vi "MAIZE Offline Console.vi"() -> ()   [LabVIEW 2025]
doc: "Offline MAIZE operator console with modeled equipment and the shared controller."
panel:
  in  "End session":bool
  out "Cryo gate valve":picture
  out "Turbo gate valve":picture
  out "Let-up valve":picture
  out "Roughing valve":picture
  out "Latched faults":string
  out "Active interlocks":string
  out "Opening outputs":string
  out "Chamber pressure":string
  out "Operating state":string
  out "Model status":string
  in  "Test condition":T1(ring)
  in  "Mode":enum16{"OFF", "MANUAL", "AUTO"}(ring)=enum."OFF"
  in  "Close / Stop":bool
  in  "Vent Start":bool
  in  "Pumpdown":bool
  in  "Arm / Reset":bool
  in  "Cryo OPEN":bool
  in  "Turbo OPEN":bool
  in  "Let-up OPEN":bool
  in  "Roughing OPEN":bool
  # "MAIZE     /     OFFLINE SIMULATION"
  # "MAINTAINED VALVE REQUESTS"
  # "Roughing and Let-up show selector requests"
  # "Turbo and Cryo show modeled reed feedback"
  # "MODE AND MOMENTARY CONTROLS"
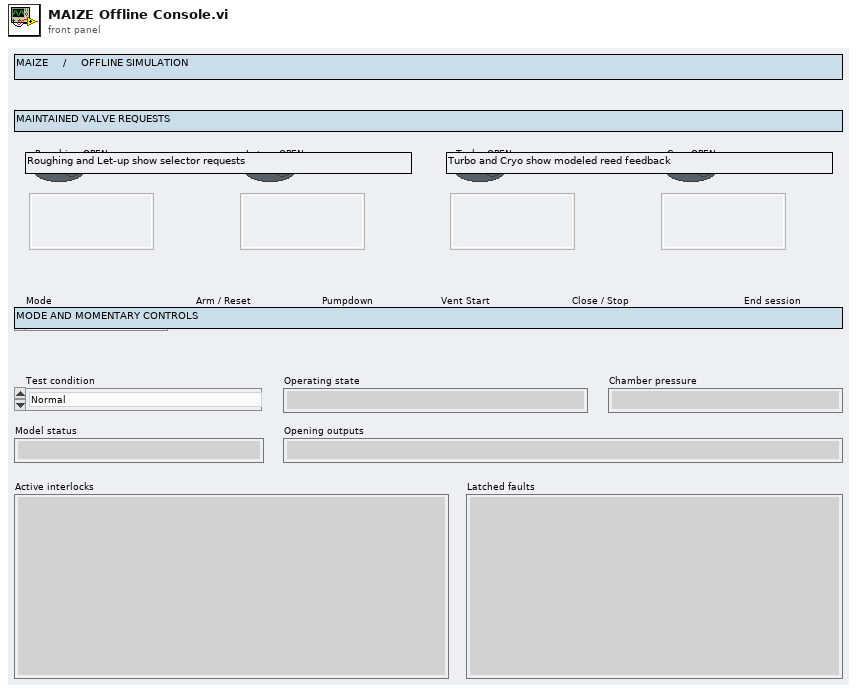
[diagram p1: front panel]
types:
  T1 = enum16{"Normal", "Pressure signal lost", "Actuator air lost", "Roughing pump not ready", "Cryopump not ready", "Turbo not at speed", "Turbo backing lost", "Filament ON", "Lab enable lost", "Coil-feed inhibit", "Vent process inhibit", "Turbo gate stuck", "Cryo gate stuck", "Turbo feedback conflict", "Cryo feedback conflict", "Panel inputs lost"}
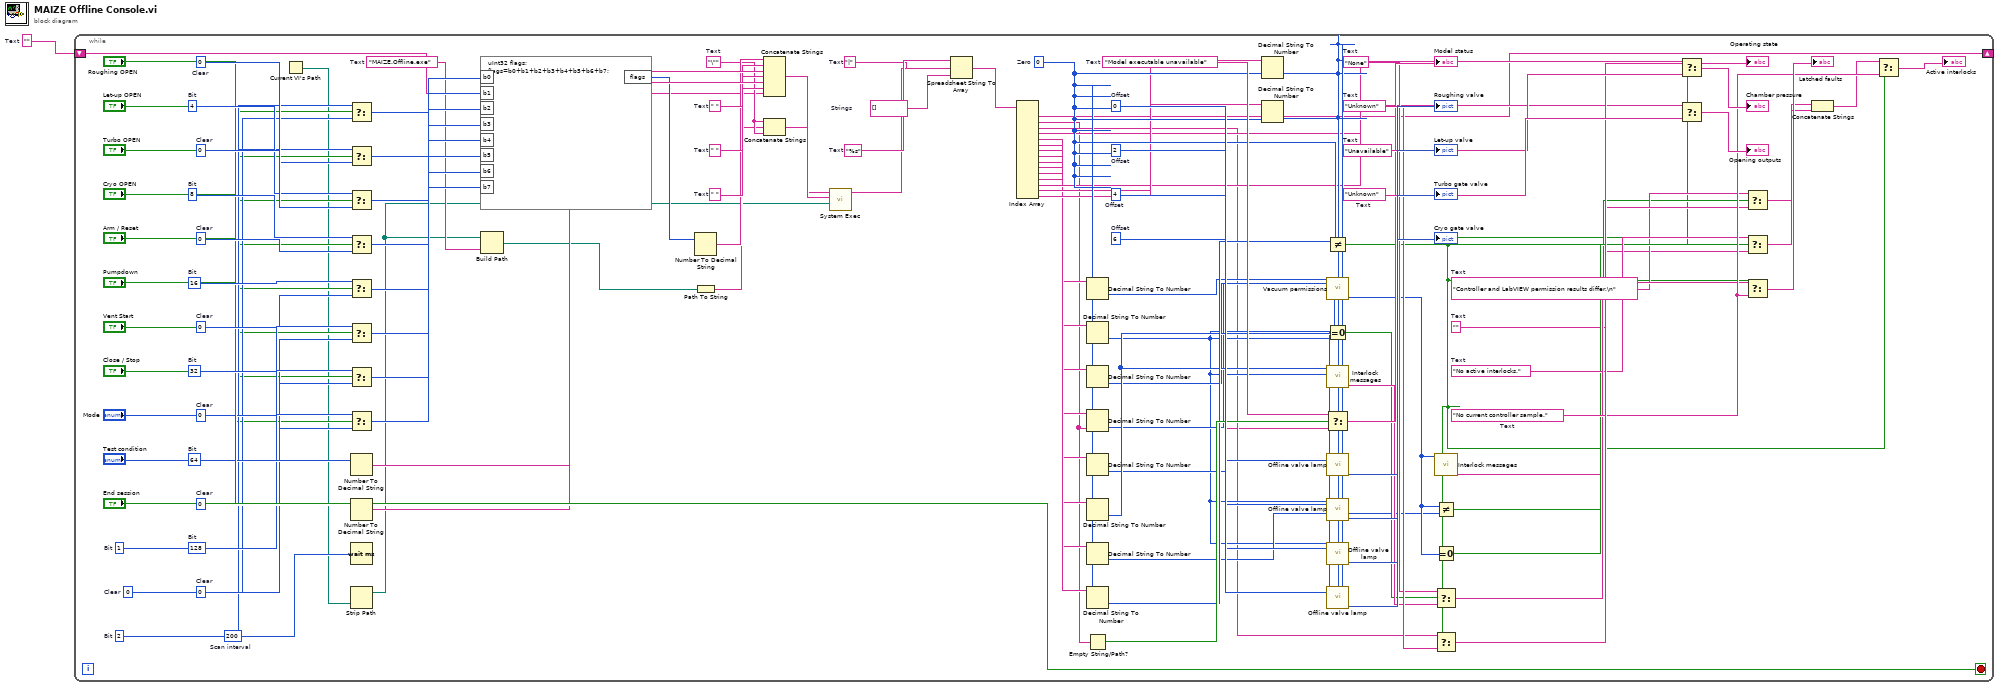
[diagram p0: block diagram]
diagram:
  w1 = ""  # Text
  n1 = while {
    shift-right: [w3] -> _
    shift-left: w1 -> [w2]
    stop <- "End session" stop-if-true
    w118 = u32 200  # Scan interval
    w116 = u32 6  # Offset
    w114 = u32 4  # Offset
    w112 = u32 2  # Offset
    w110 = u32 0  # Offset
    w104 = "Unknown"  # Text
    w102 = "Unavailable"  # Text
    w100 = "Unknown"  # Text
    w98 = "Model executable unavailable"  # Text
    w96 = "No current controller sample."  # Text
    w93 = "None"  # Text
    w89 = "No active interlocks."  # Text
    w86 = ""  # Text
    w85 = "Controller and LabVIEW permission results differ.\n"  # Text
    w72 = u32 0  # Zero
    w56 = "%s"  # Text
    w55 = string[] []  # Strings
    w54 = "|"  # Text
    w51 = " "  # Text
    w49 = " "  # Text
    w47 = " "  # Text
    w41 = u32 0  # Clear
    w40 = u32 128  # Bit
    w38 = u32 0  # Clear
    w37 = u32 64  # Bit
    w35 = u32 0  # Clear
    w34 = u32 32  # Bit
    w32 = u32 0  # Clear
    w31 = u32 16  # Bit
    w29 = u32 0  # Clear
    w28 = u32 8  # Bit
    w26 = u32 0  # Clear
    w25 = u32 4  # Bit
    w23 = u32 0  # Clear
    w22 = u32 2  # Bit
    w20 = u32 0  # Clear
    w19 = u32 1  # Bit
    w9 = "\""  # Text
    w6 = "MAIZE.Offline.exe"  # Text
    n2 = Current VI's Path() -> (path=w4:path)
    n3 = Select(t=w19, s="Roughing OPEN", f=w20) -> (s? t:f=w21:u32)
    n4 = Select(t=w22, s="Let-up OPEN", f=w23) -> (s? t:f=w24:u32)
    n5 = Select(t=w25, s="Turbo OPEN", f=w26) -> (s? t:f=w27:u32)
    n6 = Select(t=w28, s="Cryo OPEN", f=w29) -> (s? t:f=w30:u32)
    n7 = Select(t=w31, s="Arm / Reset", f=w32) -> (s? t:f=w33:u32)
    n8 = Select(t=w34, s="Pumpdown", f=w35) -> (s? t:f=w36:u32)
    n9 = Select(t=w37, s="Vent Start", f=w38) -> (s? t:f=w39:u32)
    n10 = Select(t=w40, s="Close / Stop", f=w41) -> (s? t:f=w42:u32)
    n11 = Number To Decimal String(number="Mode") -> (decimal integer string=w48:string)  [unwired: 1 in]
    n12 = Number To Decimal String(number="Test condition") -> (decimal integer string=w50:string)  [unwired: 1 in]
    n13 = Wait (ms)(milliseconds to wait=w118) -> ()  [unwired: 1 out]
    n14 = Strip Path(path=w4) -> (stripped path=w5:path)  [unwired: 1 out]
    n15 = formula code="uInt32 flags;\nflags=b0+b1+b2+b3+b4+b5+b6+b7;"("b0"=w21, "b1"=w24, "b2"=w27, "b3"=w30, "b4"=w33, "b5"=w36, "b6"=w39, "b7"=w42) -> ("flags"=w43:u32)
    n16 = Build Path(base path=w5, name or relative path=w6) -> (appended path=w7:path)
    n17 = Number To Decimal String(number=w43) -> (decimal integer string=w46:string)  [unwired: 1 in]
    n18 = Path To String(path=w7) -> (string=w8:string)
    n19 = Concatenate Strings(w46, w47, w48, w49, w50, w51, w2) -> (w52:string)
    n20 = Concatenate Strings(w9, w8, w9) -> (w10:string)
    n21 = call <vilib>:"System Exec.vi"("working directory"=w5, "standard input"=w52, "command line"=w10) -> ("standard output"=w53:string)  [unwired: 5 in, 3 out]
    n22 = Spreadsheet String To Array(delimiter (Tab)=w54, format string=w56, spreadsheet string=w53, array type (2D Dbl)=w55) -> (array=w57:string[])
    n23 = Index Array(array=w57) -> (element #1=w3:string, element #2=w58:string, element #3=w59:string, element #4=w60:string, element #5=w61:string, element #6=w62:string, element #7=w63:string, element #8=w64:string, element #9=w65:string, element #10=w66:string, element #11=w67:string, element #12=w68:string, element #13=w69:string, element #14=w70:string, element #15=w71:string)  [unwired: 15 in]
    n24 = Decimal String To Number(string=w61, default (0L)=w72) -> (number=w73:u32)  [unwired: 1 in, 1 out]
    n25 = Decimal String To Number(string=w62, default (0L)=w72) -> (number=w74:u32)  [unwired: 1 in, 1 out]
    n26 = Decimal String To Number(string=w63, default (0L)=w72) -> (number=w75:u32)  [unwired: 1 in, 1 out]
    n27 = Decimal String To Number(string=w64, default (0L)=w72) -> (number=w76:u32)  [unwired: 1 in, 1 out]
    n28 = Decimal String To Number(string=w65, default (0L)=w72) -> (number=w77:u32)  [unwired: 1 in, 1 out]
    n29 = Decimal String To Number(string=w66, default (0L)=w72) -> (number=w78:u32)  [unwired: 1 in, 1 out]
    n30 = Decimal String To Number(string=w67, default (0L)=w72) -> (number=w79:u32)  [unwired: 1 in, 1 out]
    n31 = Decimal String To Number(string=w68, default (0L)=w72) -> (number=w80:u32)  [unwired: 1 in, 1 out]
    n32 = Empty String/Path?(string/path=w58) -> (empty?=w97:bool)
    n33 = Decimal String To Number(string=w70, default (0L)=w72) -> (number=w108:u32)  [unwired: 1 in, 1 out]
    n34 = Decimal String To Number(string=w71, default (0L)=w72) -> (number=w109:u32)  [unwired: 1 in, 1 out]
    n35 = Not Equal?(x=w80, y=w72) -> (x != y?=w81:bool)
    n36 = call "Vacuum permissions.vi"("attempt"=w73, "pos"=w74, "status"=w75, "site"=w76, "events"=w77) -> ("alarms"=w82:u32)  [unwired: 10 in]
    n37 = Equal To 0?(x=w78) -> (x = 0?=w92:bool)
    n38 = call "Interlock messages.vi"("Fault bits"=w78) -> ("Messages"=w94:string)  [unwired: 14 in]
    n39 = Select(t=w98, s=w97, f=w58) -> (s? t:f=→"Model status":string)
    n40 = call "Offline valve lamp.vi"("Position word"=w74, "Bit offset"=w110, "Physical selectors"=w108, "Selector quality"=w109) -> ("Lamp"=→"Roughing valve":picture)  [unwired: 11 in]
    n41 = call "Offline valve lamp.vi"("Position word"=w74, "Bit offset"=w112, "Physical selectors"=w108, "Selector quality"=w109) -> ("Lamp"=→"Let-up valve":picture)  [unwired: 11 in]
    n42 = call "Offline valve lamp.vi"("Position word"=w74, "Bit offset"=w114, "Physical selectors"=w108, "Selector quality"=w109) -> ("Lamp"=→"Turbo gate valve":picture)  [unwired: 11 in]
    n43 = call "Offline valve lamp.vi"("Position word"=w74, "Bit offset"=w116, "Physical selectors"=w108, "Selector quality"=w109) -> ("Lamp"=→"Cryo gate valve":picture)  [unwired: 11 in]
    n44 = call "Interlock messages.vi"("Fault bits"=w82) -> ("Messages"=w83:string)  [unwired: 14 in]
    n45 = Not Equal?(x=w82, y=w79) -> (x != y?=w84:bool)
    n46 = Equal To 0?(x=w82) -> (x = 0?=w88:bool)
    n47 = Select(t=w93, s=w92, f=w94) -> (s? t:f=w95:string)
    n48 = Select(t=w59, s=w81, f=w100) -> (s? t:f=→"Operating state":string)
    n49 = Select(t=w60, s=w81, f=w102) -> (s? t:f=→"Chamber pressure":string)
    n50 = Select(t=w69, s=w81, f=w104) -> (s? t:f=→"Opening outputs":string)
    n51 = Select(t=w85, s=w84, f=w86) -> (s? t:f=w87:string)
    n52 = Select(t=w89, s=w88, f=w83) -> (s? t:f=w90:string)
    n53 = Select(t=w95, s=w81, f=w96) -> (s? t:f=→"Latched faults":string)
    n54 = Concatenate Strings(w87, w90) -> (w91:string)
    n55 = Select(t=w91, s=w81, f=w96) -> (s? t:f=→"Active interlocks":string)
  }
